vi "UI_Status_Text.vi"(0 "Settings":T1={"Sample Rate (Hz)"=1000.0, "Samples per Channel"=100, "Chassis 1 Channels"="cDAQ1Mod1/ai0:7,cDAQ1Mod2/ai0:7,cDAQ1Mod3/ai0:7,cDAQ1Mod4/ai0:7,cDAQ1Mod5/ai0:7,cDAQ1Mod6/ai0:7,cDAQ1Mod7/ai0:7,cDAQ1Mod8/ai0:7", "Chassis 2 Channels"="cDAQ2Mod1/ai0:7,cDAQ2Mod2/ai0:7,cDAQ2Mod3/ai0:7,cDAQ2Mod4/ai0:7,cDAQ2Mod5/ai0:7,cDAQ2Mod6/ai0:7,cDAQ2Mod7/ai0:7,cDAQ2Mod8/ai0:7", "Save Folder"=path "C:/LV_Test/AI DAQ md test/Data"}, 1 "Message":string, 5 "Running":bool, 7 "Logging":bool, 9 "Log File":path, 11 "error in":errorcluster) -> (4 "Status":string, 15 "error out":errorcluster)   [LabVIEW 2026]
doc: "상단 상태 문구: 측정 중/대기, 샘플링 속도, 샘플 수, 저장 파일, 메시지."
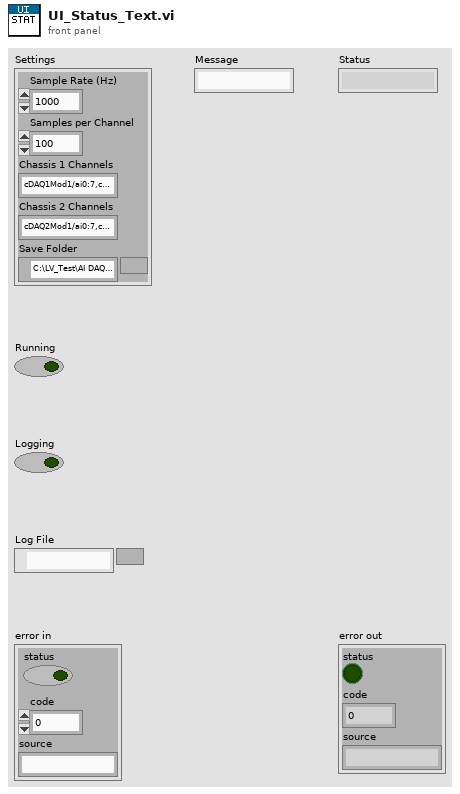
[diagram p1: front panel]
types:
  T1 = cluster{"Sample Rate (Hz)":dbl, "Samples per Channel":i32, "Chassis 1 Channels":string, "Chassis 2 Channels":string, "Save Folder":path}
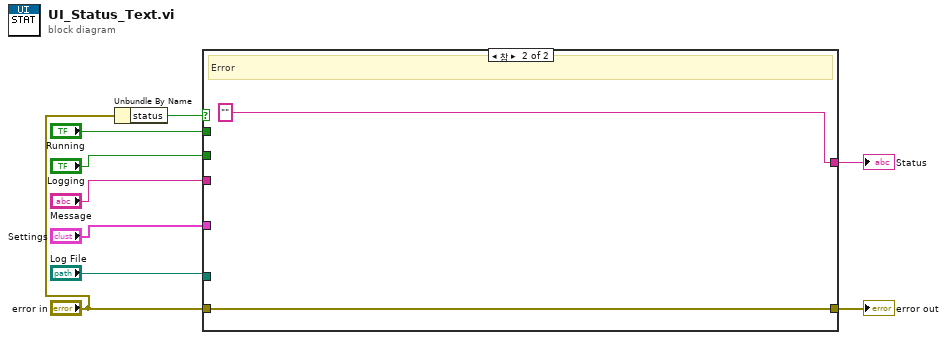
[diagram p0: block diagram]
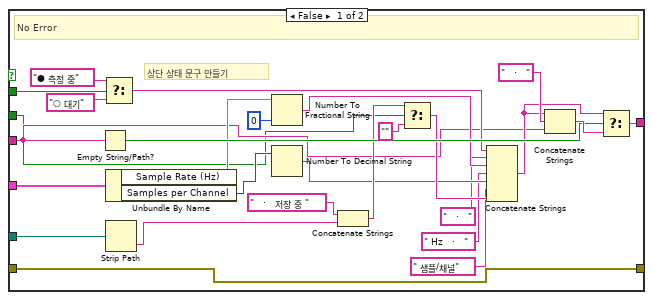
[diagram p2: hidden frame]
diagram:
  n1 = Unbundle By Name("error in") -> ("status"=w7:bool)
  n2 = case shown="참" w7 {
    tunnel: "Settings" -> [w10 _]
    tunnel: "Running" -> [w11 _]
    tunnel: "Logging" -> [w12 _]
    tunnel: "Log File" -> [w13 _]
    tunnel: "Message" -> [w14 _]
    tunnel: "error in" -> [w15 w37]
    tunnel: [w15 w37] -> w9
    tunnel: [w36 ""] -> w8
    frame False {
      # "상단 상태 문구 만들기"
      # "No Error"
      n3 = Empty String/Path?(string/path=w14) -> (empty?=w33:bool)
      n4 = Select(t="● 측정 중", s=w11, f="○ 대기") -> (s? t:f=w21:string)
      n5 = Unbundle By Name(w10) -> ("Sample Rate (Hz)"=w16:dbl, "Samples per Channel"=w17:i32)
      n6 = Strip Path(path=w13) -> (name=w18:string)  [unwired: 1 out]
      n7 = Number To Fractional String(number=w16, precision (6)=0) -> (F-format string=w24:string)  [unwired: 2 out]
      n8 = Number To Decimal String(number=w17) -> (decimal integer string=w26:string)  [unwired: 1 in]
      n9 = Concatenate Strings("   ·   저장 중 ", w18) -> (w29:string)
      n10 = Select(t=w29, s=w12, f="") -> (s? t:f=w31:string)
      n11 = Concatenate Strings(w21, "   ·   ", w24, " Hz   ·   ", w26, " 샘플/채널", w31) -> (w32:string)
      n12 = Concatenate Strings(w32, "   ·   ", w14) -> (w35:string)
      n13 = Select(t=w32, s=w33, f=w35) -> (s? t:f=w36:string)
    }
    frame True {
      # "Error"
    }
  }
  "Status" <- w8
  "error out" <- w9
